vi "Handle Server Request Batch.vi"(7 "parameters":string[][](array[string]), 8 "error in (no error)":errorcluster, 10 "id in":i32, 11 "request":string) -> (0 "error out":errorcluster, 3 "response":string)   [LabVIEW 2020, in "MCP Server.lvlib"]
doc: "Handles the body of one HTTP request, which is one JSON-RPC message or a batch of messages.\n\n- The body is a JSON array (a batch, part of the MCP protocol versions 2024-11-05 and 2025-03-26): every element is passed to Handle Server Request.vi. response is a JSON array of the answers, in the order of the messages. Notifications have no answer; if no message has an answer, response is empty. An empty array is answered with JSON-RPC error -32600 (Invalid Request) and id null.\n- Anything else, including an array that is cut off before its closing bracket, is passed to Handle Server Request.vi unchanged and response is its answer.\n\nerror out is the error out of Handle Server Request.vi for the first message."
uses:
  MCP Server.lvlib
  <vilib>/JDP Science/JSONtext/support/Format JSON Array Text.vi
  <vilib>/JDP Science/JSONtext/JSONtext.lvlib
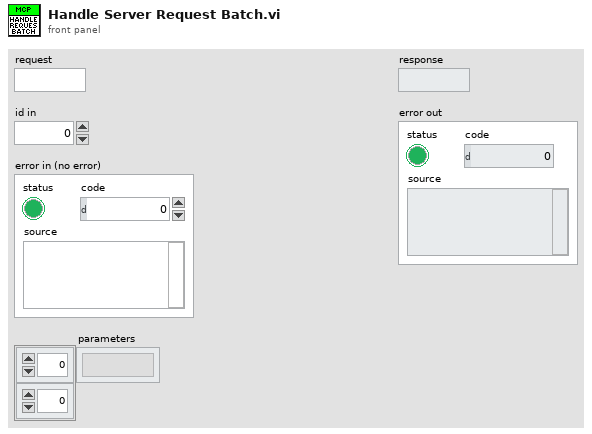
[diagram p1: front panel]
types:
  T1 = typedef "JSONtext.lvlib/JSON Value Type.ctl" = enum16{"Not a JSON Value", "JSON Object", "JSON Array", "String", "Number", "true", "false", "null"}
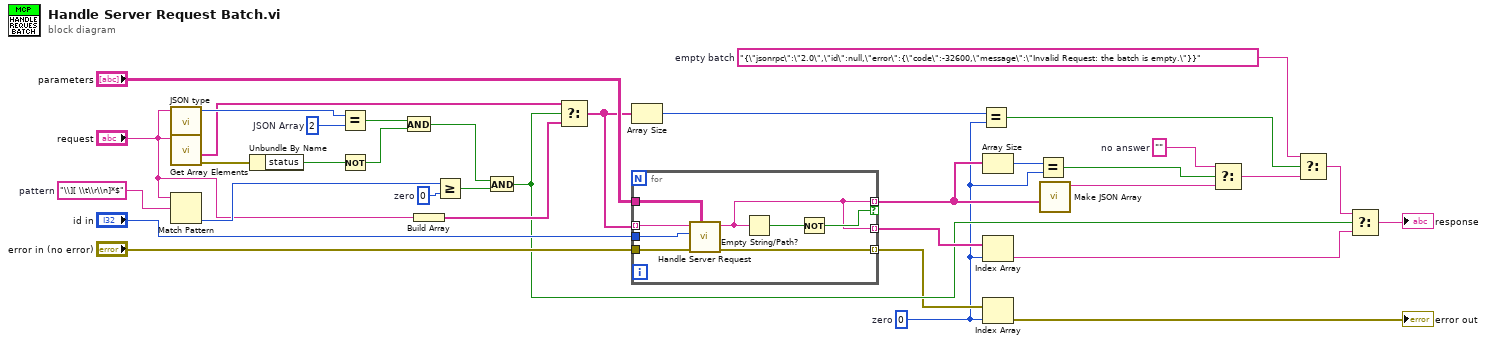
[diagram p0: block diagram]
diagram:
  w11 = "{\"jsonrpc\":\"2.0\",\"id\":null,\"error\":{\"code\":-32600,\"message\":\"Invalid Request: the batch is empty.\"}}"  # empty batch
  w15 = ""  # no answer
  w2 = 0  # zero
  w29 = 0  # zero
  w31 = "\\][ \\t\\r\\n]*$"  # pattern
  w34 = u16 2  # JSON Array
  n1 = call <vilib>:"JSON type.vi"("JSON"="request") -> ("JSON Value Type"=w35:T1)  [unwired: 9 in, 1 out]
  n2 = call <vilib>:"Get Array Elements.vi"("JSON"="request") -> ("error out"=w33:errorcluster, "<JSON>"=w23:string[])  [unwired: 8 in, 1 out]
  n3 = Match Pattern(string="request", regular expression=w31) -> (offset past match=w30:i32)  [unwired: 1 in, 3 out]
  n4 = Unbundle By Name(w33) -> ("status"=w32:bool)
  n5 = Equal?(x=w35, y=w34) -> (x = y?=w28:bool)
  n6 = Not(x=w32) -> (.not. x?=w27:bool)
  n7 = And(x=w28, y=w27) -> (x .and. y?=w26:bool)
  n8 = Build Array("request") -> (w22:string[])
  n9 = Greater Or Equal?(x=w30, y=w29) -> (x >= y?=w25:bool)
  n10 = And(x=w26, y=w25) -> (x .and. y?=w6:bool)
  n11 = Select(t=w23, s=w6, f=w22) -> (s? t:f=w18:string[])
  n12 = Array Size(array=w18) -> (size(s)=w12:i32)
  n13 = for {
    tunnel: w18 -> [w43] mode=indexing
    tunnel: "id in" -> [w42]
    tunnel: "parameters" -> [w40]
    tunnel: "error in (no error)" -> [w41]
    tunnel: [w37] -> w8 mode=indexing
    tunnel: [w37] -> w16 mode=indexing if=w38
    tunnel: [w36] -> w3 mode=indexing
    n14 = call "Handle Server Request.vi"("parameters"=w40, "error in (no error)"=w41, "id in"=w42, "request"=w43) -> ("error out"=w36:errorcluster, "response"=w37:string)  [unwired: 6 in]
    n15 = Empty String/Path?(string/path=w37) -> (empty?=w39:bool)
    n16 = Not(x=w39) -> (.not. x?=w38:bool)
  }
  n17 = Equal?(x=w12, y=w2) -> (x = y?=w10:bool)
  n18 = Array Size(array=w16) -> (size(s)=w17:i32)
  n19 = Index Array(array=w8, index=w2) -> (element=w5:string)
  n20 = Index Array(array=w3, index=w2) -> (element=→"error out":errorcluster)
  n21 = Equal?(x=w17, y=w2) -> (x = y?=w14:bool)
  n22 = call <vilib>:"Make JSON Array.vi"("JSON Elements"=w16) -> ("<JSON>"=w13:string)  [unwired: 9 in, 1 out]
  n23 = Select(t=w15, s=w14, f=w13) -> (s? t:f=w9:string)
  n24 = Select(t=w11, s=w10, f=w9) -> (s? t:f=w7:string)
  n25 = Select(t=w7, s=w6, f=w5) -> (s? t:f=→"response":string)
